vi "StoreTestEventsOnRunIDFolder.vi"(8 "error in":errorcluster, 11 "Events array":T1[](array[typedef])=[{"Test Instruction"="1. Install the Icon Editor.", "Sample Number"=8, "Relative seconds"=680.3219987, "Frame Number"=0}, {"Test Instruction"="2. Open Icon Editor Manual Tests.lvproj.", "Sample Number"=4638, "Relative seconds"=704.0259920999999, "Frame Number"=56}, {"Test Instruction"="3. Open and run Remove Icon Editor Settings.vi. This ensures there are no Icon Editor keys in the LabVIEW.ini file. All of the key names start with \"IconEditor.\"", "Sample Number"=8959, "Relative seconds"=728.0703004, "Frame Number"=343}, {"Test Instruction"="4. Close the VI and project.", "Sample Number"=11193, "Relative seconds"=739.3449462, "Frame Number"=479}, {"Test Instruction"="", "Sample Number"=12440, "Relative seconds"=745.6403978, "Frame Number"=554}, {"Test Instruction"="1. Open a new VI from the Getting Started Window.", "Sample Number"=13484, "Relative seconds"=750.9241820999999, "Frame Number"=617}, {"Test Instruction"="2. From the Front Panel, double-click on the VI Icon.", "Sample Number"=16600, "Relative seconds"=766.8371073, "Frame Number"=809}]) -> (0 "error out":errorcluster)   [LabVIEW 2026, in "testCoordinator.lvlib"]
uses:
  testCoordinator.lvlib
  modules/coordinator/src/Libraries/Core/global.vi
  modules/coordinator/src/Libraries/Launcher/Launcher.lvlib
  6b591763-2b5e-4d96-80b1-b01cc2295bc4.vi
  modules/coordinator/src/Libraries/UserEventRecorder/TestEvent.ctl
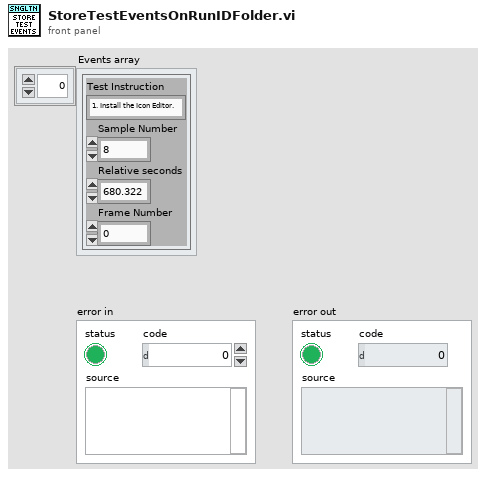
[diagram p1: front panel]
types:
  T1 = typedef "TestEvent.ctl" = cluster{"Test Instruction":string, "Sample Number":u32, "Relative seconds":dbl, "Frame Number":u32}
  T2 = enum16{"open", "replace", "create", "open or create", "replace or create", "replace or create with confirmation"}
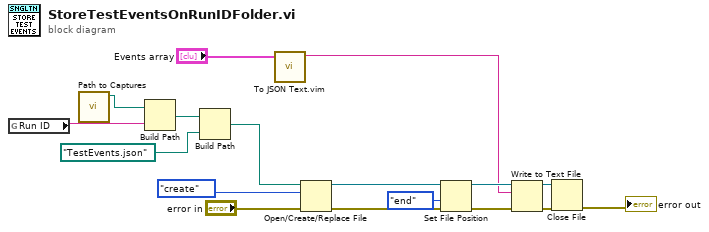
[diagram p0: block diagram]
diagram:
  n1 = global read "global.vi" "Run ID"() -> (w7:string)
  n2 = call "Path to Captures.vi"() -> ("Captures"=w8:path)  [unwired: 11 in]
  n3 = Build Path(base path=w8, name or relative path=w7) -> (appended path=w6:path)
  n4 = Build Path(base path=w6, name or relative path=path "TestEvents.json") -> (appended path=w3:path)
  n5 = call "To JSON Text.vim"("Anything"="Events array") -> ("<JSON>"=w1:string)  [unwired: 9 in, 1 out]
  n6 = Open/Create/Replace File(file path (use dialog)=w3, error in="error in", operation (0:open)=T2."create") -> (refnum out=w17:refnum<file>, error out=w16:errorcluster)  [unwired: 3 in, 1 out]
  n7 = Set File Position(refnum=w17, from (0:start)=enum16{"start", "end", "current"}."end", error in=w16) -> (refnum out=w14:refnum<file>, error out=w15:errorcluster)  [unwired: 1 in]
  n8 = Write to Text File(file (use dialog)=w14, text=w1, error in=w15) -> (refnum out=w12:refnum<file>, error out=w11:errorcluster)  [unwired: 1 in, 1 out]
  n9 = Close File(refnum=w12, error in=w11) -> (error out=→"error out":errorcluster)  [unwired: 1 out]
